vi "KYFG Camera Start Acquire.vi"(8 "error in (no error)":errorcluster, 9 "frames":u32, 10 "buffHandle":u32, 11 "camHandle":u32) -> (0 "error out":errorcluster, 2 "buffHandle out":u32, 3 "camHandle out":u32)   [LabVIEW 2023, in "KYFGLib_lv.lvlib"]
doc: "KYFG_API FGSTATUS KYFG_CameraStartAcquire(CAMHANDLE camHandle, BUFFHANDLE buffHandle, unsigned int frames);"
uses:
  KYFGLib_lv.lvlib
  KYFGLib.dll
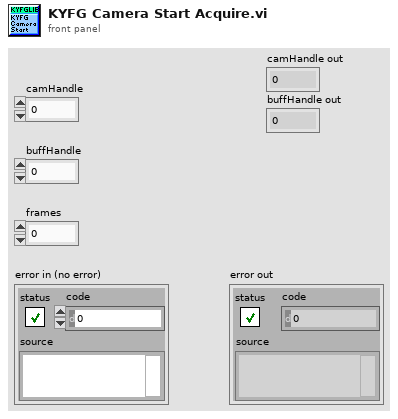
[diagram p1: front panel]
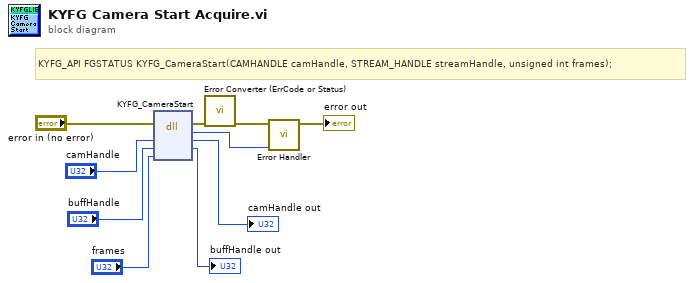
[diagram p0: block diagram]
diagram:
  # "KYFG_API FGSTATUS KYFG_CameraStart(CAMHANDLE camHandle, STREAM_HANDLE streamHandle, unsigned int frames);"
  n1 = dll-call lib="KYFGLib.dll" fn="KYFG_CameraStart"(error in="error in (no error)", "camHandle"="camHandle", "streamHandle"="buffHandle", "frames"="frames") -> (error out=w6:errorcluster, "return type"=w3:u32, "camHandle"=→"camHandle out":u32, "streamHandle"=→"buffHandle out":u32)  [unwired: 3 in, 1 out]
  n2 = call "Error Converter (ErrCode or Status).vi"("error in (no error)"=w6) -> ("error out"=w5:errorcluster)  [unwired: 10 in]
  n3 = call "Error Handler.vi"("Return Code"=w3, "Error In"=w5) -> ("Error Out"=→"error out":errorcluster)  [unwired: 9 in]
